vi "Write Save Path.vi"(8 "error in (no error)":errorcluster, 10 "Save Path":path, 11 "Abstract DAQ Triggered Actor in":refnum<class "Abstract DAQ Triggered Actor.lvclass">) -> (0 "error out":errorcluster, 3 "Abstract DAQ Triggered Actor out":refnum<class "Abstract DAQ Triggered Actor.lvclass">)   [LabVIEW 2020, in "DAQ Timed SPIM.lvlib" / "Abstract DAQ Triggered Actor.lvlib" / "Abstract DAQ Triggered Actor.lvclass"]
uses:
  Abstract DAQ Triggered Actor.lvclass
  Abstract DAQ Triggered Actor.lvclass/Abstract DAQ Triggered Actor.ctl
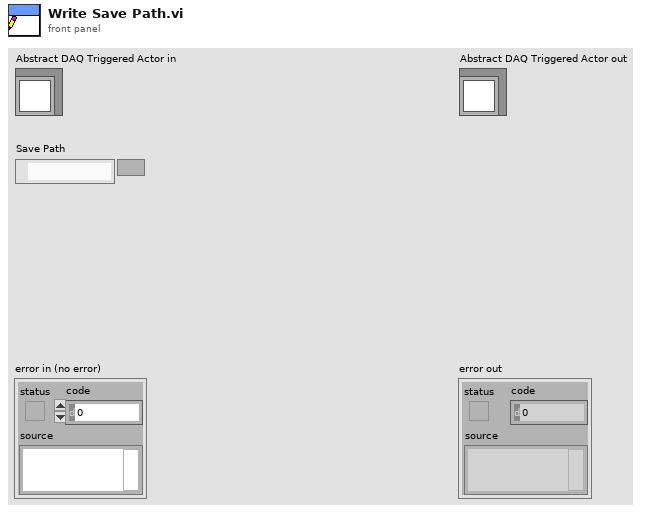
[diagram p1: front panel]
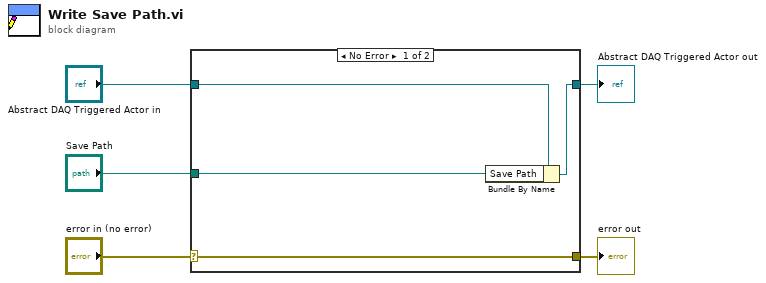
[diagram p0: block diagram]
diagram:
  n1 = case shown="No Error" "error in (no error)" {
    selector: "error in (no error)" -> [w9 w10]
    tunnel: [w9 w10] -> w4
    tunnel: [w7 w11] -> w2
    tunnel: "Abstract DAQ Triggered Actor in" -> [w8 w11]
    tunnel: "Save Path" -> [w6 _]
    frame No Error {
      n2 = Bundle By Name(cluster=w8, "Save Path"=w6) -> (w7:refnum<class "Abstract DAQ Triggered Actor.lvclass">)
    }
    frame Error {
    }
  }
  "error out" <- w4
  "Abstract DAQ Triggered Actor out" <- w2
